vi "Read Interface_Spectrum.lvclass.vi"(8 "error in (no error)":errorcluster, 11 "Band Edge in":refnum<class "Band Edge.lvclass">) -> (0 "error out":errorcluster, 2 "Interface_Spectrum.lvclass":refnum<class "Interface_Spectrum.lvclass">, 3 "Band Edge out":refnum<class "Band Edge.lvclass">)   [LabVIEW 2023, in "Spectrum Analyzer.lvlib" / "Band Edge.lvclass"]
uses:
  Band Edge.lvclass
  Band Edge.lvclass/Band Edge.ctl
  Interface_Spectrum/Interface_Spectrum.lvclass
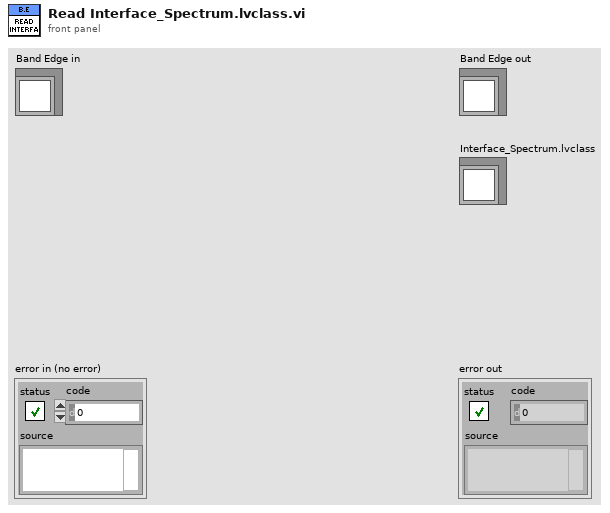
[diagram p1: front panel]
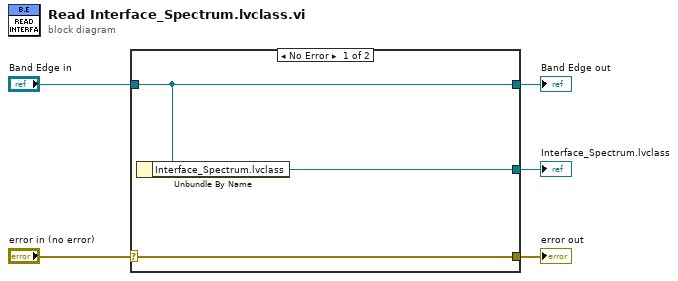
[diagram p0: block diagram]
diagram:
  n1 = case shown="No Error" "error in (no error)" {
    selector: "error in (no error)" -> [w8 w9]
    tunnel: [w8 w9] -> w4
    tunnel: [w7 w10] -> w2
    tunnel: "Band Edge in" -> [w7 w10]
    tunnel: [w6 _] -> w1
    frame No Error {
      n2 = Unbundle By Name(w7) -> ("Interface_Spectrum.lvclass"=w6:refnum<class "Interface_Spectrum.lvclass">)
    }
    frame Error {
    }
  }
  "error out" <- w4
  "Band Edge out" <- w2
  "Interface_Spectrum.lvclass" <- w1
